vi "initalization.vi"(8 "error in (no error)":errorcluster) -> (0 "error out":errorcluster)   [LabVIEW 2019]
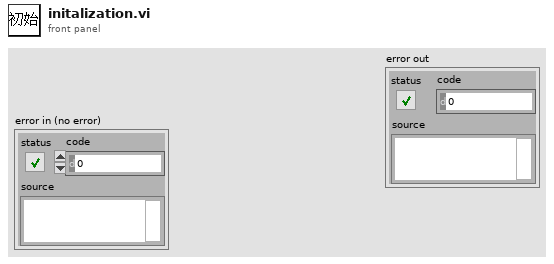
[diagram p1: front panel]
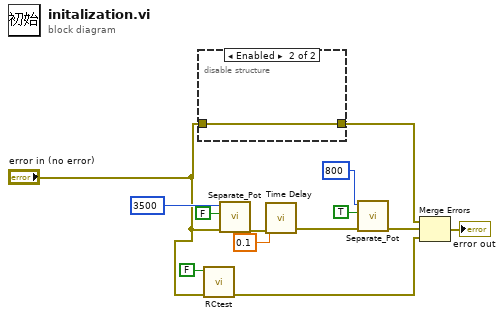
[diagram p0: block diagram]
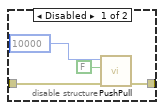
[diagram p2: hidden frame]
diagram:
  n1 = disable-structure shown="Enabled" {
    disable-tunnel: "error in (no error)" -> [w15 w18]
    disable-tunnel: [w14 w18] -> w9
    frame Disabled {
      n2 = call "PushPull.vi"("error in (no error)"=w15, "轉向"=FALSE, "距離"=10000) -> ("error out"=w14:errorcluster)  [unwired: 7 in, 1 out]
    }
    frame Enabled {
    }
  }
  n3 = call "RCtest.vi"("error in (no error)"="error in (no error)", "s"=FALSE) -> ("error out"=w8:errorcluster)  [unwired: 9 in]
  n4 = call "Separate_Pot.vi"("error in (no error)"="error in (no error)", "轉向"=FALSE, "距離"=3500) -> ("error out"=w6:errorcluster)  [unwired: 7 in, 1 out]
  n5 = call "Time Delay"("error in (no error)"=w6, "Delay Time (s)"=0.1) -> ("error out"=w5:errorcluster)  [unwired: 9 in]
  n6 = call "Separate_Pot.vi"("error in (no error)"=w5, "轉向"=TRUE, "距離"=800) -> ("error out"=w4:errorcluster)  [unwired: 7 in, 1 out]
  n7 = Merge Errors(w9, w4, w8) -> (→"error out":errorcluster)
